vi "GT_Log.vi"(8 "error in (no error)":errorcluster, 9 "Text":string, 10 "Code":u16, 11 "Event":string) -> (3 "error out":errorcluster)   [LabVIEW 2026]
doc: "Use this template to build a VI to use as a subVI."
uses:
  <vilib>/Utility/file.llb/Write Delimited Spreadsheet (string).vi
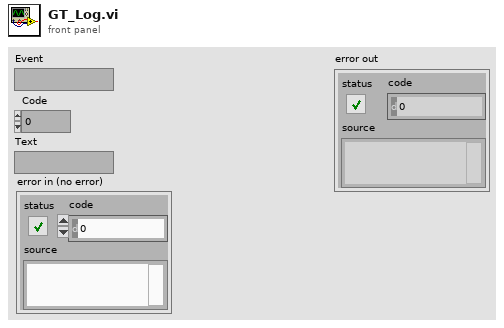
[diagram p1: front panel]
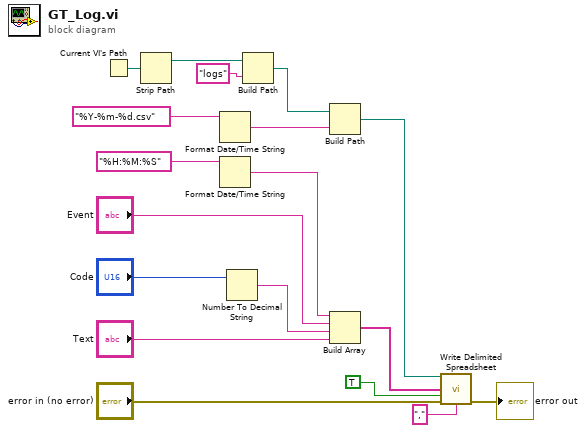
[diagram p0: block diagram]
diagram:
  n1 = Current VI's Path() -> (path=w18:path)
  n2 = Strip Path(path=w18) -> (stripped path=w17:path)  [unwired: 1 out]
  n3 = Format Date/Time String(time format string (%c)="%Y-%m-%d.csv") -> (date/time string=w13:string)  [unwired: 2 in]
  n4 = Format Date/Time String(time format string (%c)="%H:%M:%S") -> (date/time string=w10:string)  [unwired: 2 in]
  n5 = Number To Decimal String(number="Code") -> (decimal integer string=w8:string)  [unwired: 1 in]
  n6 = Build Path(base path=w17, name or relative path="logs") -> (appended path=w14:path)
  n7 = Build Path(base path=w14, name or relative path=w13) -> (appended path=w6:path)
  n8 = Build Array(w10, "Event", w8, "Text") -> (w5:string[])
  n9 = call-poly <vilib>:"Write Delimited Spreadsheet.vi"("file path (dialog if empty)"=w6, "1D data"=w5, "append to file? (new file:F)"=TRUE, "error in (no error)"="error in (no error)", "delimiter (\\t)"=",") -> ("error out"=→"error out":errorcluster)  [unwired: 9 in, 1 out]
